vi "HolDrvCtrl_Execute.vi"(0 "Period":dbl=0.02, 4 "Rot Vel Feedforward\nRad/Sec":dbl, 5 "HOLONOMIC_CTRL_PACK_TUNING":T1={"X PID Tuning"={"Kp"=0.0, "Ki"=0.0, "Kd"=0.0, "MaximumIntegral"=9.9e+30, "MinimumIntegral"=-9.9e+30, "IntegralZone"=9.9e+30}, "Y PID Tuning"={"Kp"=0.0, "Ki"=0.0, "Kd"=0.0, "MaximumIntegral"=9.9e+30, "MinimumIntegral"=-9.9e+30, "IntegralZone"=9.9e+30}, "thetaProfiledPID_CTRL"={"Controller"={"Kp"=0.0, "Ki"=0.0, "Kd"=0.0, "Period"=0.0, "Max_Integral"=1.0, "Min_Integral"=-1.0, "Max_Input"=0.0, "Min_Input"=0.0, "Continuous"=FALSE, "PositionError"=0.0, "VelocityError"=0.0, "PrevError"=0.0, "Total_Integral"=0.0, "PositionTolerance"=0.05, "VelocityTolerance"=9.99e+35, "SetPoint"=0.0, "Kf"=0.0, "Prev_Deriv"=0.0, "Prev_Deriv 2"=0.0, "DerivativeFilter"=FALSE, "Min_Output"=-9.99e+35, "Max_Output"=9.9e+35, "Prev_F_P"=0.0, "Prev_F_P_2"=0.0, "AntiWindupActive"=FALSE, "Measurement"=0.0, "IntegralZone"=9.9e+30}, "Goal"={"Position"=0.0, "Velocity"=0.0}, "Setpoint"={"Position"=0.0, "Velocity"=0.0}, "Constraint"={"MaxVelocity"=0.0, "MaxAcceleration"=0.0}}} {"thetaProfiledPID_CTRL"."Constraint"."MaxAcceleration" format="%16_6e"; "thetaProfiledPID_CTRL"."Constraint"."MaxVelocity" format="%16_6e"; "thetaProfiledPID_CTRL"."Setpoint"."Velocity" format="%16_6e"; "thetaProfiledPID_CTRL"."Setpoint"."Position" format="%16_6e"; "thetaProfiledPID_CTRL"."Goal"."Velocity" format="%16_6e"; "thetaProfiledPID_CTRL"."Goal"."Position" format="%16_6e"; "thetaProfiledPID_CTRL"."Controller"."IntegralZone" format="%16_6e"; "thetaProfiledPID_CTRL"."Controller"."Measurement" format="%16_6e"; "thetaProfiledPID_CTRL"."Controller"."Prev_F_P_2" format="%16_6e"; "thetaProfiledPID_CTRL"."Controller"."Prev_F_P" format="%16_6e"; "thetaProfiledPID_CTRL"."Controller"."Max_Output" format="%16_6e"; "thetaProfiledPID_CTRL"."Controller"."Min_Output" format="%16_6e"; "thetaProfiledPID_CTRL"."Controller"."Prev_Deriv 2" format="%16_6e"; "thetaProfiledPID_CTRL"."Controller"."Prev_Deriv" format="%16_6e"; "thetaProfiledPID_CTRL"."Controller"."Kf" format="%16_6e"; "thetaProfiledPID_CTRL"."Controller"."SetPoint" format="%16_6e"; "thetaProfiledPID_CTRL"."Controller"."VelocityTolerance" format="%16_6e"; "thetaProfiledPID_CTRL"."Controller"."PositionTolerance" format="%16_6e"; "thetaProfiledPID_CTRL"."Controller"."Total_Integral" format="%16_6e"; "thetaProfiledPID_CTRL"."Controller"."PrevError" format="%16_6e"; "thetaProfiledPID_CTRL"."Controller"."VelocityError" format="%16_6e"; "thetaProfiledPID_CTRL"."Controller"."PositionError" format="%16_6e"; "thetaProfiledPID_CTRL"."Controller"."Min_Input" format="%16_6e"; "thetaProfiledPID_CTRL"."Controller"."Max_Input" format="%16_6e"; "thetaProfiledPID_CTRL"."Controller"."Min_Integral" format="%16_6e"; "thetaProfiledPID_CTRL"."Controller"."Max_Integral" format="%16_6e"; "thetaProfiledPID_CTRL"."Controller"."Period" format="%16_6e"; "thetaProfiledPID_CTRL"."Controller"."Kd" format="%16_6e"; "thetaProfiledPID_CTRL"."Controller"."Ki" format="%16_6e"; "thetaProfiledPID_CTRL"."Controller"."Kp" format="%16_6e"}, 6 "Reset":bool, 7 "Tolerance":T7={"TRANSLATION"={"X"=0.04, "Y"=0.04}, "ROTATION"={"VALUE"=0.034906585039887, "COS"=0.999390827019096, "SIN"=0.034899496702501}} {"ROTATION"."SIN" format="%13.4f"; "ROTATION"."COS" format="%13.4f"; "ROTATION"."VALUE" format="%13.4f"; "TRANSLATION"."Y" format="%14.3f"; "TRANSLATION"."X" format="%14.3f"}, 8 "Enable":bool=TRUE, 9 "angleRef":T9={"VALUE"=0.0, "COS"=1.0, "SIN"=0.0} {"SIN" format="%13.4f"; "COS" format="%13.4f"; "VALUE" format="%13.4f"}, 10 "HolExecuteSP":cluster{"out POSe":T7, "LinearVel":dbl} {"out POSe"."ROTATION"."SIN" format="%13.4f"; "out POSe"."ROTATION"."COS" format="%13.4f"; "out POSe"."ROTATION"."VALUE" format="%13.4f"; "out POSe"."TRANSLATION"."Y" format="%14.3f"; "out POSe"."TRANSLATION"."X" format="%14.3f"}, 11 "currentPose":T7={"TRANSLATION"={"X"=0.0, "Y"=0.0}, "ROTATION"={"VALUE"=0.0, "COS"=1.0, "SIN"=0.0}} {"ROTATION"."SIN" format="%13.4f"; "ROTATION"."COS" format="%13.4f"; "ROTATION"."VALUE" format="%13.4f"; "TRANSLATION"."Y" format="%14.3f"; "TRANSLATION"."X" format="%14.3f"}) -> (1 "outHOLONOMIC_DRV_CTRL":T11={"poseTolerance"={"TRANSLATION"={"X"=0.0, "Y"=0.0}, "ROTATION"={"VALUE"=0.0, "COS"=1.0, "SIN"=0.0}}, "poseError"={"TRANSLATION"={"X"=0.0, "Y"=0.0}, "ROTATION"={"VALUE"=0.0, "COS"=1.0, "SIN"=0.0}}, "Enabled"=TRUE, "PID_xCtrl"={"Kp"=0.0, "Ki"=0.0, "Kd"=0.0, "Period"=0.0, "Max_Integral"=1.0, "Min_Integral"=-1.0, "Max_Input"=0.0, "Min_Input"=0.0, "Continuous"=FALSE, "PositionError"=0.0, "VelocityError"=0.0, "PrevError"=0.0, "Total_Integral"=0.0, "PositionTolerance"=0.05, "VelocityTolerance"=9.99e+35, "SetPoint"=0.0, "Kf"=0.0, "Prev_Deriv"=0.0, "Prev_Deriv 2"=0.0, "DerivativeFilter"=FALSE, "Min_Output"=-9.99e+35, "Max_Output"=9.9e+35, "Prev_F_P"=0.0, "Prev_F_P_2"=0.0, "AntiWindupActive"=FALSE, "Measurement"=0.0, "IntegralZone"=9.9e+30}, "PID_yCtrl"={"Kp"=0.0, "Ki"=0.0, "Kd"=0.0, "Period"=0.0, "Max_Integral"=1.0, "Min_Integral"=-1.0, "Max_Input"=0.0, "Min_Input"=0.0, "Continuous"=FALSE, "PositionError"=0.0, "VelocityError"=0.0, "PrevError"=0.0, "Total_Integral"=0.0, "PositionTolerance"=0.05, "VelocityTolerance"=9.99e+35, "SetPoint"=0.0, "Kf"=0.0, "Prev_Deriv"=0.0, "Prev_Deriv 2"=0.0, "DerivativeFilter"=FALSE, "Min_Output"=-9.99e+35, "Max_Output"=9.9e+35, "Prev_F_P"=0.0, "Prev_F_P_2"=0.0, "AntiWindupActive"=FALSE, "Measurement"=0.0, "IntegralZone"=9.9e+30}, "PROF_PID_thetaCtrl"={"Controller"={"Kp"=0.0, "Ki"=0.0, "Kd"=0.0, "Period"=0.0, "Max_Integral"=1.0, "Min_Integral"=-1.0, "Max_Input"=0.0, "Min_Input"=0.0, "Continuous"=FALSE, "PositionError"=0.0, "VelocityError"=0.0, "PrevError"=0.0, "Total_Integral"=0.0, "PositionTolerance"=0.05, "VelocityTolerance"=9.99e+35, "SetPoint"=0.0, "Kf"=0.0, "Prev_Deriv"=0.0, "Prev_Deriv 2"=0.0, "DerivativeFilter"=FALSE, "Min_Output"=-9.99e+35, "Max_Output"=9.9e+35, "Prev_F_P"=0.0, "Prev_F_P_2"=0.0, "AntiWindupActive"=FALSE, "Measurement"=0.0, "IntegralZone"=9.9e+30}, "Goal"={"Position"=0.0, "Velocity"=0.0}, "Setpoint"={"Position"=0.0, "Velocity"=0.0}, "Constraint"={"MaxVelocity"=0.0, "MaxAcceleration"=0.0}}, "RotationError"={"VALUE"=0.0, "COS"=1.0, "SIN"=0.0}, "FirstRun"=FALSE} {"RotationError"."SIN" format="%13.4f"; "RotationError"."COS" format="%13.4f"; "RotationError"."VALUE" format="%13.4f"; "PROF_PID_thetaCtrl"."Constraint"."MaxAcceleration" format="%16_6e"; "PROF_PID_thetaCtrl"."Constraint"."MaxVelocity" format="%16_6e"; "PROF_PID_thetaCtrl"."Setpoint"."Velocity" format="%16_6e"; "PROF_PID_thetaCtrl"."Setpoint"."Position" format="%16_6e"; "PROF_PID_thetaCtrl"."Goal"."Velocity" format="%16_6e"; "PROF_PID_thetaCtrl"."Goal"."Position" format="%16_6e"; "PROF_PID_thetaCtrl"."Controller"."IntegralZone" format="%16_6e"; "PROF_PID_thetaCtrl"."Controller"."Measurement" format="%16_6e"; "PROF_PID_thetaCtrl"."Controller"."Prev_F_P_2" format="%16_6e"; "PROF_PID_thetaCtrl"."Controller"."Prev_F_P" format="%16_6e"; "PROF_PID_thetaCtrl"."Controller"."Max_Output" format="%16_6e"; "PROF_PID_thetaCtrl"."Controller"."Min_Output" format="%16_6e"; "PROF_PID_thetaCtrl"."Controller"."Prev_Deriv 2" format="%16_6e"; "PROF_PID_thetaCtrl"."Controller"."Prev_Deriv" format="%16_6e"; "PROF_PID_thetaCtrl"."Controller"."Kf" format="%16_6e"; "PROF_PID_thetaCtrl"."Controller"."SetPoint" format="%16_6e"; "PROF_PID_thetaCtrl"."Controller"."VelocityTolerance" format="%16_6e"; "PROF_PID_thetaCtrl"."Controller"."PositionTolerance" format="%16_6e"; "PROF_PID_thetaCtrl"."Controller"."Total_Integral" format="%16_6e"; "PROF_PID_thetaCtrl"."Controller"."PrevError" format="%16_6e"; "PROF_PID_thetaCtrl"."Controller"."VelocityError" format="%16_6e"; "PROF_PID_thetaCtrl"."Controller"."PositionError" format="%16_6e"; "PROF_PID_thetaCtrl"."Controller"."Min_Input" format="%16_6e"; "PROF_PID_thetaCtrl"."Controller"."Max_Input" format="%16_6e"; "PROF_PID_thetaCtrl"."Controller"."Min_Integral" format="%16_6e"; "PROF_PID_thetaCtrl"."Controller"."Max_Integral" format="%16_6e"; "PROF_PID_thetaCtrl"."Controller"."Period" format="%16_6e"; "PROF_PID_thetaCtrl"."Controller"."Kd" format="%16_6e"; "PROF_PID_thetaCtrl"."Controller"."Ki" format="%16_6e"; "PROF_PID_thetaCtrl"."Controller"."Kp" format="%16_6e"; "PID_yCtrl"."IntegralZone" format="%16_6e"; "PID_yCtrl"."Measurement" format="%16_6e"; "PID_yCtrl"."Prev_F_P_2" format="%16_6e"; "PID_yCtrl"."Prev_F_P" format="%16_6e"; "PID_yCtrl"."Max_Output" format="%16_6e"; "PID_yCtrl"."Min_Output" format="%16_6e"; "PID_yCtrl"."Prev_Deriv 2" format="%16_6e"; "PID_yCtrl"."Prev_Deriv" format="%16_6e"; "PID_yCtrl"."Kf" format="%16_6e"; "PID_yCtrl"."SetPoint" format="%16_6e"; "PID_yCtrl"."VelocityTolerance" format="%16_6e"; "PID_yCtrl"."PositionTolerance" format="%16_6e"; "PID_yCtrl"."Total_Integral" format="%16_6e"; "PID_yCtrl"."PrevError" format="%16_6e"; "PID_yCtrl"."VelocityError" format="%16_6e"; "PID_yCtrl"."PositionError" format="%16_6e"; "PID_yCtrl"."Min_Input" format="%16_6e"; "PID_yCtrl"."Max_Input" format="%16_6e"; "PID_yCtrl"."Min_Integral" format="%16_6e"; "PID_yCtrl"."Max_Integral" format="%16_6e"; "PID_yCtrl"."Period" format="%16_6e"; "PID_yCtrl"."Kd" format="%16_6e"; "PID_yCtrl"."Ki" format="%16_6e"; "PID_yCtrl"."Kp" format="%16_6e"; "PID_xCtrl"."IntegralZone" format="%16_6e"; "PID_xCtrl"."Measurement" format="%16_6e"; "PID_xCtrl"."Prev_F_P_2" format="%16_6e"; "PID_xCtrl"."Prev_F_P" format="%16_6e"; "PID_xCtrl"."Max_Output" format="%16_6e"; "PID_xCtrl"."Min_Output" format="%16_6e"; "PID_xCtrl"."Prev_Deriv 2" format="%16_6e"; "PID_xCtrl"."Prev_Deriv" format="%16_6e"; "PID_xCtrl"."Kf" format="%16_6e"; "PID_xCtrl"."SetPoint" format="%16_6e"; "PID_xCtrl"."VelocityTolerance" format="%16_6e"; "PID_xCtrl"."PositionTolerance" format="%16_6e"; "PID_xCtrl"."Total_Integral" format="%16_6e"; "PID_xCtrl"."PrevError" format="%16_6e"; "PID_xCtrl"."VelocityError" format="%16_6e"; "PID_xCtrl"."PositionError" format="%16_6e"; "PID_xCtrl"."Min_Input" format="%16_6e"; "PID_xCtrl"."Max_Input" format="%16_6e"; "PID_xCtrl"."Min_Integral" format="%16_6e"; "PID_xCtrl"."Max_Integral" format="%16_6e"; "PID_xCtrl"."Period" format="%16_6e"; "PID_xCtrl"."Kd" format="%16_6e"; "PID_xCtrl"."Ki" format="%16_6e"; "PID_xCtrl"."Kp" format="%16_6e"; "poseError"."ROTATION"."SIN" format="%13.4f"; "poseError"."ROTATION"."COS" format="%13.4f"; "poseError"."ROTATION"."VALUE" format="%13.4f"; "poseError"."TRANSLATION"."Y" format="%14.3f"; "poseError"."TRANSLATION"."X" format="%14.3f"; "poseTolerance"."ROTATION"."SIN" format="%13.4f"; "poseTolerance"."ROTATION"."COS" format="%13.4f"; "poseTolerance"."ROTATION"."VALUE" format="%13.4f"; "poseTolerance"."TRANSLATION"."Y" format="%14.3f"; "poseTolerance"."TRANSLATION"."X" format="%14.3f"}, 2 "AtReference":bool, 3 "calcChassisSpeed":T10 {"vOmega" format="%10.3f"; "vY" format="%10.3f"; "vX" format="%10.3f"})   [LabVIEW 2019, in "Trajectory_Library.lvlib"]
doc: "This holonomic drive controller can be used to follow trajectories using a holonomic drivetrain (i.e. swerve or mecanum). Holonomic trajectory following is a much simpler problem to solve compared to skid-steer style drivetrains because it is possible to individually control forward, sideways, and angular velocity.\n\nThe holonomic drive controller takes in one PID controller for each direction, forward and sideways, and one profiled PID controller for the angular direction. Because the heading dynamics are decoupled from translations, users can specify a custom heading that the drivetrain should point toward. This heading reference is profiled for smoothness.\n\nThis convience function creates and executes a Holonomic Controller. It uses a packed Setpoint (SP), created by the HolDrvCtrl_PackSP.vi, as the setping and the current pose as the process variable. It returns a chassis speed as the control utput.\n\nNOTE: This version does not support dynamic tuning. All the unint inputs and Tolerance are used only on the first call.\n \nInputs:\n - X PID Tuning - Input from PACK PROF PID VI\n - Y PID Tuning - Input from PACK PROF PID VI\n - thetaController -- A profiled PID controller to respond to error in angle.\n - CurrentPose -- Current location\n -HolExecuteSP -- Desired location and speed cluster. This contains:\n - Desired Pose -- X,Y,Heading\n - Linear Velocity -- Desired velocity\n - AngleRef -- Current angle of orientation.\n - Enable -- Enable close loop control. If disabled, the feedforwards from the trajectory state are used.\n - Period -- Execution period (Default 0.020) Seconds.\n - Tolerance -- Amount of position and heading error allowed to be considered on target. (Default 0.04, 0.04, 0.034)\n\nOutputs:\n - ChassisSpeed -- ChassisSpeed setpoint calcuated from the inputs.\n - AtTarget -- Boolean indicating the position and heading are within the provided tolerance.\n - HolonomicDriveController -- Data structure (can be used for debug or extracting information)"
uses:
  Trajectory_Library.lvlib
  TypeDef/HOLONOMIC_DRV_CTRL.ctl
  TypeDef/POSE2D.ctl
  TypeDef/TRANSLATION2D.ctl
  TypeDef/ROTATION2D.ctl
  TypeDef/PID_CONTROLLER.ctl
  TypeDef/PROFILED_PID_CONTROLLER.ctl
  TypeDef/TRAPEZOID_PROFILE_STATE.ctl
  TypeDef/TRAPEZOID_PROFILE_CONSTRAINT.ctl
  TypeDef/CHASSIS_SPEEDS.ctl
  TypeDef/HOLONOMIC_PACK_TUNING.ctl
  TypeDef/PID_TUNING.ctl
  ProfiledPIDController_EnableContInput.vi
  Conv_Deg_Radians.vi
  PIDController_NewPeriod.vi
  PIDController_SetIntegratorRange.vi
  PIDController_Reset.vi
  Pose2d_getXYAngle.vi
  Rotation2d_GetRadians.vi
  Rotation2d_GetAngleCosSin.vi
  Pose2d_RelativeTo.vi
  Pose2d_getRotation.vi
  Rotation2d_Minus.vi
  ProfiledPIDController_Calculate_Meas_Goal.vi
  PIDController_Calculate_SP_PV.vi
  ProfiledPIDController_Reset_PosOnly.vi
  ChassisSpeeds_FromFieldRelativeSpeeds.vi
  PIDController_EnableContinousInput.vi
  <vilib>/Rock Robotics/SystemInterfaces/NetworkCommunication/NetComm_UsageReport_report.vi
  Transform2d_Create_PosePose.vi
  Pose2d_New_TRRO.vi
  Rotation2d_UnaryMinus.vi
  Rotation2d_RotateBy.vi
  ProfiledPIDController_SetGoal_PosOnly.vi
  ProfiledPIDController_Calculate_Meas.vi
  PIDController_SetSetpoint.vi
  PIDController_Calculate_PV.vi
  TrapProfState_New.vi
  ProfiledPIDController_Reset.vi
  Rotation2d_GetCos.vi
  Rotation2d_GetSin.vi
  ChassisSpeeds_New.vi
  Translation2d_RotateBy.vi
  Translation2d_Minus.vi
  Rotation2d_CreateAngle.vi
  Rotation2d_CreateXY.vi
  ProfiledPIDController_SetGoal.vi
  TrapProfile_New.vi
  ProfiledPIDController_GetPeriod.vi
  TrapProfile_Calculate.vi
  ControllerUtil_GetModulusError.vi
  Translation2d_Create.vi
  Util_CalcDist.vi
  TrapProfile_ShouldFlipAcceleration.vi
  TrapProfile_Direct.vi
  PIDController_GetPeriod.vi
  Globals/Util_LibraryGlobals.vi
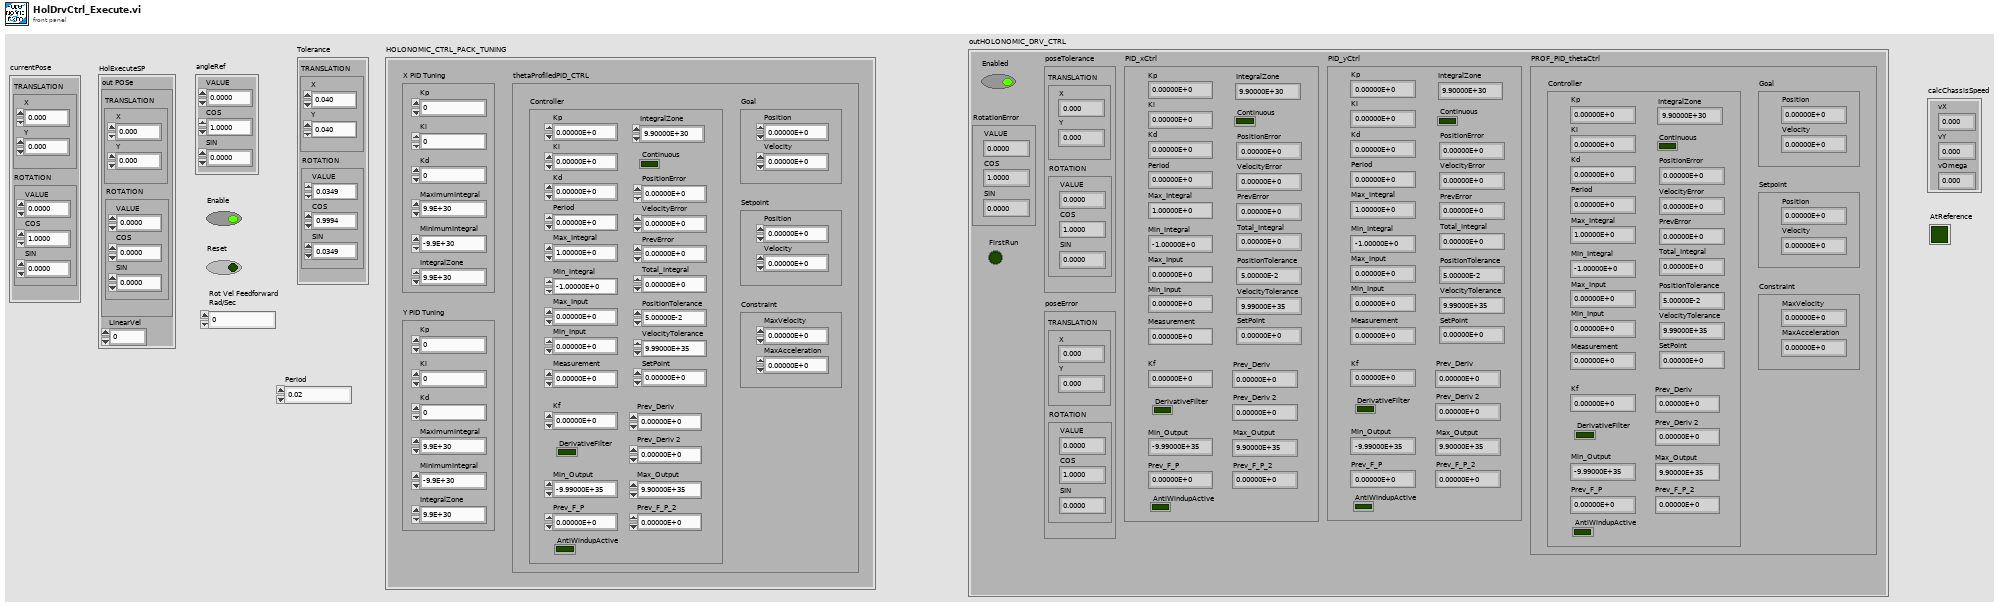
[diagram p1: front panel]
types:
  T1 = typedef "Trajectory_Library.lvlib/HOLONOMIC_PACK_TUNING.ctl" = cluster{"X PID Tuning":T2, "Y PID Tuning":T2, "thetaProfiledPID_CTRL":T3}
  T2 = typedef "Trajectory_Library.lvlib/PID_TUNING.ctl" = cluster{"Kp":dbl, "Ki":dbl, "Kd":dbl, "MaximumIntegral":dbl, "MinimumIntegral":dbl, "IntegralZone":dbl}
  T3 = typedef "Trajectory_Library.lvlib/PROFILED_PID_CONTROLLER.ctl" = cluster{"Controller":T4, "Goal":T5, "Setpoint":T5, "Constraint":T6}
  T4 = typedef "Trajectory_Library.lvlib/PID_CONTROLLER.ctl" = cluster{"Kp":dbl, "Ki":dbl, "Kd":dbl, "Period":dbl, "Max_Integral":dbl, "Min_Integral":dbl, "Max_Input":dbl, "Min_Input":dbl, "Continuous":bool, "PositionError":dbl, "VelocityError":dbl, "PrevError":dbl, "Total_Integral":dbl, "PositionTolerance":dbl, "VelocityTolerance":dbl, "SetPoint":dbl, "Kf":dbl, "Prev_Deriv":dbl, "Prev_Deriv 2":dbl, "DerivativeFilter":bool, "Min_Output":dbl, "Max_Output":dbl, "Prev_F_P":dbl, "Prev_F_P_2":dbl, "AntiWindupActive":bool, "Measurement":dbl, "IntegralZone":dbl}
  T5 = typedef "Trajectory_Library.lvlib/TRAPEZOID_PROFILE_STATE.ctl" = cluster{"Position":dbl, "Velocity":dbl}
  T6 = typedef "Trajectory_Library.lvlib/TRAPEZOID_PROFILE_CONSTRAINT.ctl" = cluster{"MaxVelocity":dbl, "MaxAcceleration":dbl}
  T7 = typedef "Trajectory_Library.lvlib/POSE2D.ctl" = cluster{"TRANSLATION":T8, "ROTATION":T9}
  T8 = typedef "Trajectory_Library.lvlib/TRANSLATION2D.ctl" = cluster{"X":dbl, "Y":dbl}
  T9 = typedef "Trajectory_Library.lvlib/ROTATION2D.ctl" = cluster{"VALUE":dbl, "COS":dbl, "SIN":dbl}
  T10 = typedef "Trajectory_Library.lvlib/CHASSIS_SPEEDS.ctl" = cluster{"vX":dbl, "vY":dbl, "vOmega":dbl}
  T11 = typedef "Trajectory_Library.lvlib/HOLONOMIC_DRV_CTRL.ctl" = cluster{"poseTolerance":T7, "poseError":T7, "Enabled":bool, "PID_xCtrl":T4, "PID_yCtrl":T4, "PROF_PID_thetaCtrl":T3, "RotationError":T9, "FirstRun":bool}
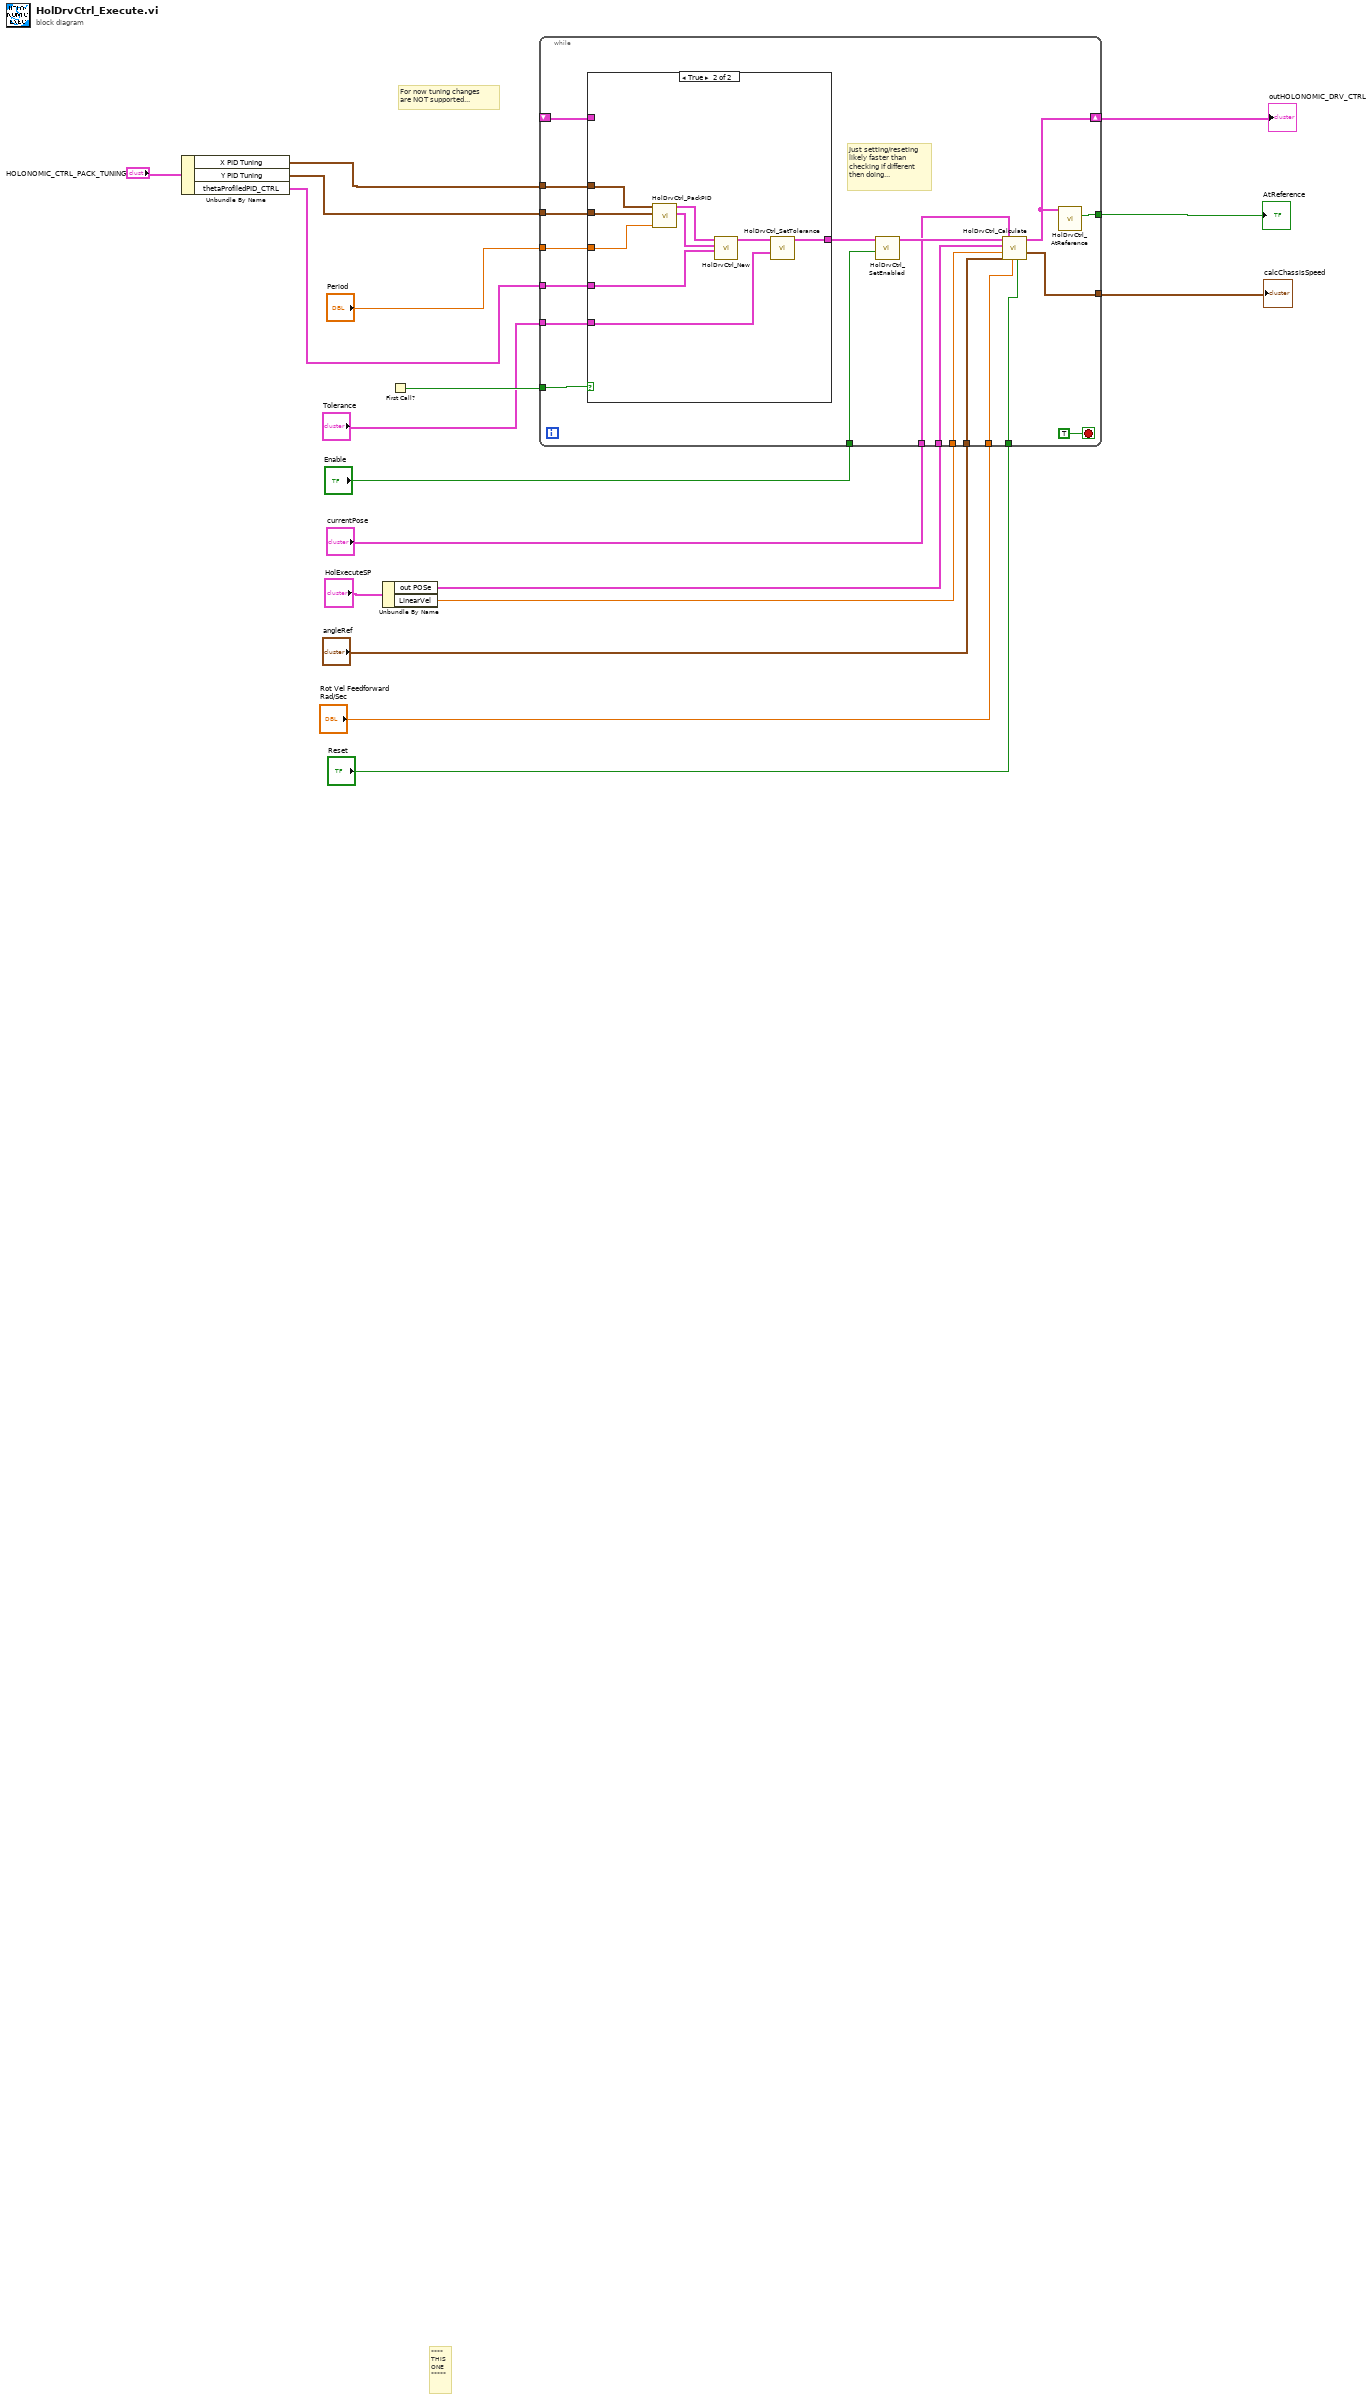
[diagram p0: block diagram]
diagram:
  # "For now tuning changes\nare NOT supported..."
  # "****\nTHIS\nONE\n*****"
  n1 = Unbundle By Name("HOLONOMIC_CTRL_PACK_TUNING") -> ("X PID Tuning"=w5:T2, "Y PID Tuning"=w4:T2, "thetaProfiledPID_CTRL"=w3:T3)
  n2 = Unbundle By Name("HolExecuteSP") -> ("out POSe"=w8:T7, "LinearVel"=w7:dbl)
  n3 = First Call?() -> (First Call?: T/F=w18:bool)
  n4 = while {
    tunnel: w18 -> [w38]
    tunnel: w3 -> [w37]
    tunnel: "Enable" -> [w35]
    tunnel: "currentPose" -> [w33]
    tunnel: "angleRef" -> [w32]
    tunnel: [w31] -> w14
    tunnel: w5 -> [w30]
    tunnel: w4 -> [w29]
    tunnel: "Period" -> [w28]
    shift-right: [w24] -> w12
    shift-left: _ -> [w26]
    tunnel: [w25] -> w11
    tunnel: "Tolerance" -> [w23]
    tunnel: w8 -> [w22]
    tunnel: w7 -> [w21]
    tunnel: "Rot Vel Feedforward\nRad/Sec" -> [w20]
    tunnel: "Reset" -> [w19]
    stop <- TRUE stop-if-true
    # "Just setting/reseting\nlikely faster than\nchecking if different\nthen doing..."
    n5 = case shown="True" w38 {
      tunnel: w37 -> [_ w48]
      tunnel: [w39 w40] -> w36
      tunnel: w30 -> [_ w45]
      tunnel: w29 -> [_ w44]
      tunnel: w28 -> [_ w43]
      tunnel: w26 -> [w39 _]
      tunnel: w23 -> [_ w42]
      frame False {
        # "#TODO Check for tuning\nchanges and update..."
      }
      frame True {
        n6 = call "HolDrvCtrl_PackPID.vi"("Period"=w43, "Y PID Tuning"=w44, "X PID Tuning"=w45) -> ("Y PID CONTROLLER"=w46:T4, "X PID_CONTROLLER"=w47:T4)  [unwired: 7 in]
        n7 = call "HolDrvCtrl_New.vi"("thetaProfiledPID_CTRL"=w48, "yPID_CTRL"=w46, "xPID_CTRL"=w47) -> ("outHOLONOMIC_DRV_CTRL"=w41:T11)  [unwired: 8 in]
        n8 = call "HolDrvCtrl_SetTolerance.vi"("poseTolerance"=w42, "inHOLONOMIC_DRV_CTRL"=w41) -> ("outHOLONOMIC_DRV_CTRL"=w40:T11)  [unwired: 9 in]
      }
    }
    n9 = call "HolDrvCtrl_SetEnabled.vi"("Enabled"=w35, "inHOLONOMIC_DRV_CTRL"=w36) -> ("outHOLONOMIC_DRV_CTRL"=w34:T11)  [unwired: 9 in]
    n10 = call "HolDrvCtrl_Calculate.vi"("Reset"=w19, "Rotational Vel\nFF Rad/Sec"=w20, "currentPose"=w33, "desiredHeading"=w32, "desiredLinearVelocity\nMetersPerSecond"=w21, "trajectoryPose"=w22, "inHOLONOMIC_DRV_CTRL"=w34) -> ("calcChassisSpeed"=w31:T10, "outHOLONOMIC_DRV_CTRL"=w24:T11)  [unwired: 3 in]
    n11 = call "HolDrvCtrl_AtReference.vi"("HOLONOMIC_DRV_CTRL"=w24) -> ("AtReference"=w25:bool)  [unwired: 10 in]
  }
  "outHOLONOMIC_DRV_CTRL" <- w12
  "calcChassisSpeed" <- w14
  "AtReference" <- w11
